vi "Queue-Push Element.vi"(8 "error in":errorcluster, 10 "element":variant, 11 "Buffer in":refnum<data-value>) -> (0 "error out":errorcluster, 1 "overflowed":bool, 2 "overflow":variant, 3 "Buffer":refnum<data-value>, 4 "full":bool)   [LabVIEW 2013, in "CircularBuffer.lvlib" / "VariantBuffer.lvclass"]
doc: "This VI writes one data element into the current location in the buffer. The location in the buffer is updated automatically."
uses:
  VariantBuffer.lvclass
  buffer-errors -- ring.ctl
  VariantBuffer.lvclass/VariantBuffer.ctl
  buffer-event -- enum.ctl
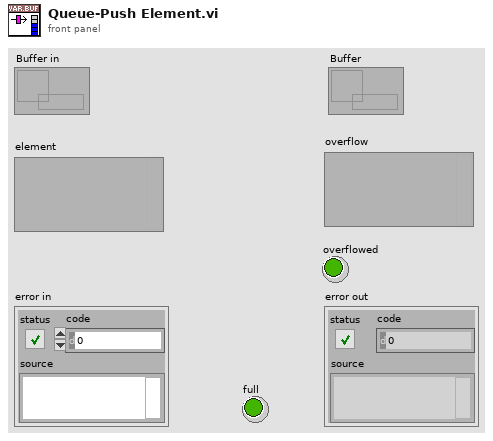
[diagram p1: front panel]
types:
  T1 = typedef "CircularBuffer.lvlib/VariantBuffer.lvclass/buffer-errors -- ring.ctl" = i32
  T2 = typedef "CircularBuffer.lvlib/VariantBuffer.lvclass/buffer-type -- enum.ctl" = enum16{"Queue", "Stack"}
  T3 = typedef "CircularBuffer.lvlib/VariantBuffer.lvclass/buffer-event -- enum.ctl" = enum16{"element-added", "element-removed", "filled", "emptied", "resized", "default-changed", "destroyed"}
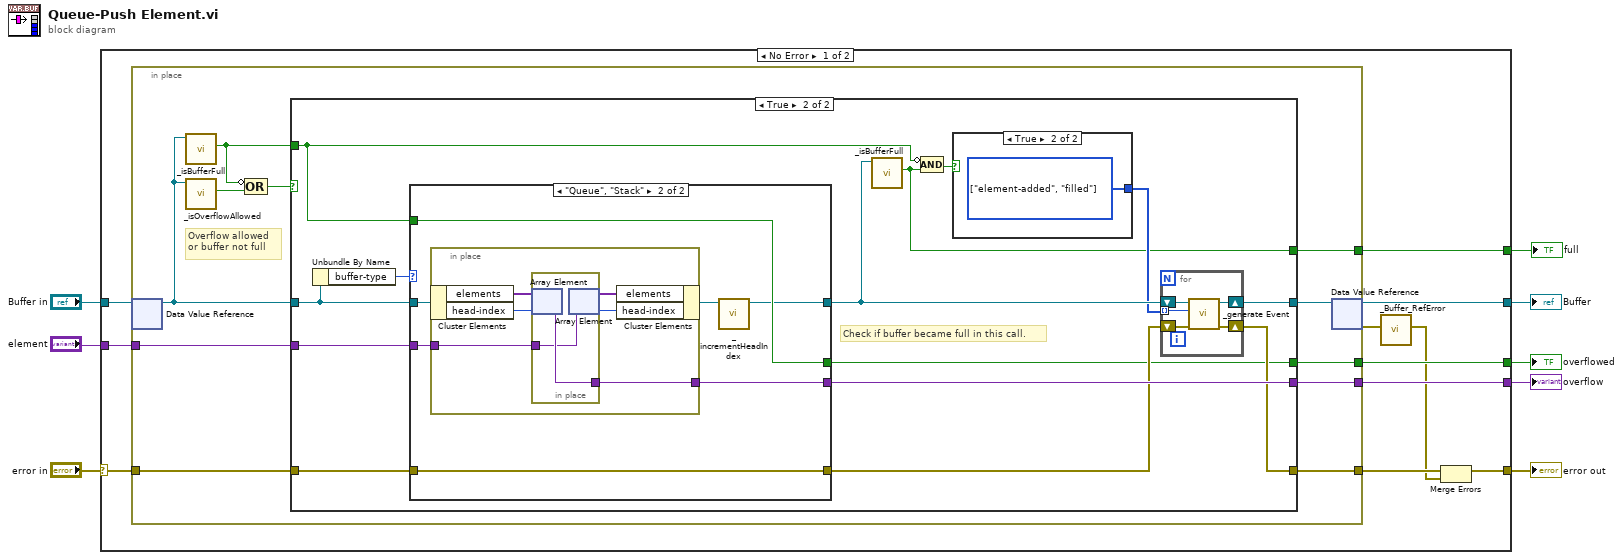
[diagram p0: block diagram]
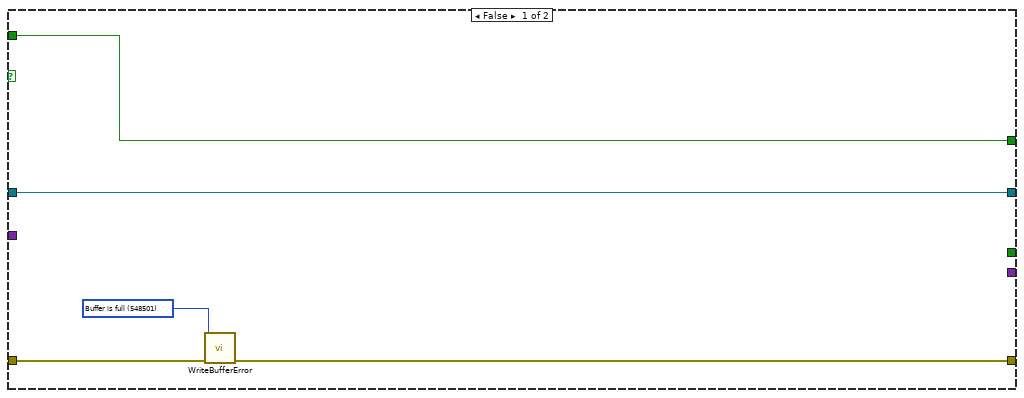
[diagram p2: hidden frame]
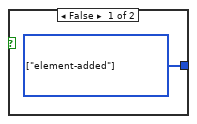
[diagram p3: hidden frame]
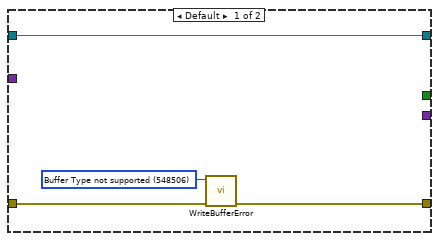
[diagram p4: hidden frame]
diagram:
  n1 = case shown="No Error" "error in" {
    selector: "error in" -> [w13 w77]
    tunnel: "Buffer in" -> [w19 w76]
    tunnel: [w16 w76] -> w7
    tunnel: [w18 w77] -> w6
    tunnel: "element" -> [w17 _]
    tunnel: [w15 _] -> w3
    tunnel: [w14 _] -> w2
    tunnel: [w9 _] -> w1
    frame No Error {
      n2 = in-place {
        in-place-border: w17 -> [w30]
        in-place-border: [w29] -> w15
        in-place-border: [w28] -> w14
        in-place-border: w13 -> [w24]
        in-place-border: [w23] -> w12
        in-place-border: [w20] -> w9
        # "Overflow allowed\nor buffer not full"
        n3 = in-place-dvr #1(w19) -> (w27:refnum<class "VariantBuffer.lvclass">)  [unwired: 1 out]
        n4 = call "_isBufferFull.vi"("VariantBuffer in"=w27) -> ("isFull"=w22:bool)  [unwired: 10 in]
        n5 = call "_isOverflowAllowed.vi"("VariantBuffer in"=w27) -> ("Allow Overflow?"=w21:bool)  [unwired: 10 in]
        n6 = Compound Arithmetic op=OR(invert w22, w21) -> (w26:bool)
        n7 = case shown="True" w26 {
          tunnel: w30 -> [_ w49]
          tunnel: [w33 w44] -> w25
          tunnel: [_ w48] -> w29
          tunnel: [_ w37] -> w28
          tunnel: w27 -> [w33 w47]
          tunnel: w24 -> [w35 w45]
          tunnel: [w34 w43] -> w23
          tunnel: w22 -> [w31 w38]
          tunnel: [w31 w36] -> w20
          frame False {
            w32 = T1 548501 items=["No error"=0, "Generic Buffer error"=548500, "Buffer is full"=548501, "Buffer is empty"=548502, "Buffer size cannot be 0"=548503, "Buffer reference is invalid"=548504, "Buffer event reference invalid"=548505] ("buffer-errors")
            n8 = call "WriteBufferError.vi"("error in (no error)"=w35, "buffer-errors"=w32) -> ("error out"=w34:errorcluster)  [unwired: 9 in]
          }
          frame True {
            # "Check if buffer became full in this call."
            n9 = Unbundle By Name(w47) -> ("buffer-type"=w46:T2)
            n10 = case shown="\"Queue\", \"Stack\"" w46 {
              tunnel: w49 -> [_ w67]
              tunnel: [_ w66] -> w48
              tunnel: [_ w63] -> w37
              tunnel: w47 -> [w60 w65]
              tunnel: [w60 w61] -> w41
              tunnel: [w58 w64] -> w42
              tunnel: w45 -> [w59 w64]
              tunnel: w38 -> [_ w63]
              frame Default {
                w57 = T1 548506 items=["No error"=0, "Generic Buffer error"=548500, "Buffer is full"=548501, "Buffer is empty"=548502, "Buffer size cannot be 0"=548503, "Buffer reference is invalid"=548504, "Buffer event reference invalid"=548505, "Buffer Type not supported"=548506] ("buffer-errors")
                n11 = call "WriteBufferError.vi"("error in (no error)"=w59, "buffer-errors"=w57) -> ("error out"=w58:errorcluster)  [unwired: 9 in]
              }
              frame "Queue", "Stack" {
                n12 = in-place {
                  in-place-border: w67 -> [w72]
                  in-place-border: [w69] -> w66
                  n13 = in-place-cluster #2(w65) -> ("elements"=w73:variant[], "head-index"=w70:i32)
                  n14 = in-place {
                    in-place-border: w72 -> [w74]
                    in-place-border: [w75] -> w69
                    n15 = in-place-array #3(w73, w70) -> (w75:variant)
                    n16 = in-place-array #3(w74) -> (w71:variant[], w68:i32)
                  }
                  n17 = in-place-cluster #2("elements"=w71, "head-index"=w68) -> (w62:refnum<class "VariantBuffer.lvclass">)
                }
                n18 = call "_incrementHeadIndex.vi"("VariantBuffer in"=w62) -> ("VariantBuffer out"=w61:refnum<class "VariantBuffer.lvclass">)  [unwired: 10 in]
              }
            }
            n19 = call "_isBufferFull.vi"("VariantBuffer in"=w41) -> ("isFull"=w36:bool)  [unwired: 10 in]
            n20 = Compound Arithmetic op=AND(invert w38, w36) -> (w40:bool)
            n21 = case shown="True" w40 {
              tunnel: [w50 w51] -> w39
              frame False {
                w50 = T3[] [enum."element-added"] items=["element-added", "element-removed", "filled", "emptied", "resized", "default-changed", "destroyed"]
              }
              frame True {
                w51 = T3[] [enum."element-added", enum."filled"] items=["element-added", "element-removed", "filled", "emptied", "resized", "default-changed", "destroyed"]
              }
            }
            n22 = for {
              tunnel: w39 -> [w54] mode=indexing
              shift-right: [w56] -> w44
              shift-left: w41 -> [w55]
              shift-right: [w53] -> w43
              shift-left: w42 -> [w52]
              n23 = call "_generate Event.vi"("error in"=w52, "event"=w54, "VariantBuffer"=w55) -> ("error out"=w53:errorcluster, "VariantBuffer out"=w56:refnum<class "VariantBuffer.lvclass">)  [unwired: 7 in]
            }
          }
        }
        n24 = in-place-dvr #1(w25) -> (w16:refnum<data-value>, w11:errorcluster)
      }
      n25 = call "_Buffer_RefError.vi"("error in (no error)"=w11) -> ("error out"=w10:errorcluster)  [unwired: 10 in]
      n26 = Merge Errors(w12, w10) -> (w18:errorcluster)
    }
    frame Error {
    }
  }
  "error out" <- w6
  "Buffer" <- w7
  "overflow" <- w3
  "overflowed" <- w2
  "full" <- w1
